vi "Get Rx Label Configuration.vi"(8 "error in":errorcluster, 10 "configuration string":string, 11 "port ref":T1 format="%.0x") -> (0 "error out":errorcluster, 2 "configuration string out":string, 3 "port ref out":T1 format="%.0x")   [LabVIEW 2020, in "Ballard ARINC 429 Hardware Configuration.lvlib"]
uses:
  Ballard ARINC 429 Hardware Configuration.lvlib
  <vilib>/NI VeriStand/Custom Device API/Custom Device Item Ref.ctl
  Constants.vi
  Scripting/Ballard/Ballard ARINC 429 Scripting.lvlib
  <vilib>/NI VeriStand/Custom Device API/Custom Device API.lvlib
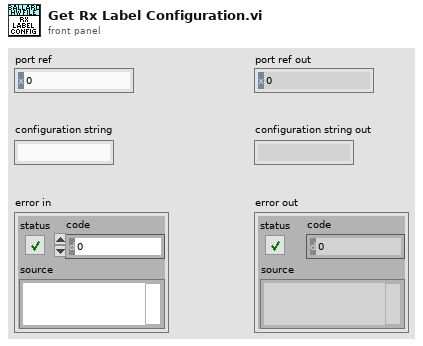
[diagram p1: front panel]
types:
  T1 = typedef "Custom Device API.lvlib/Custom Device Item Ref.ctl" = u64
  T2 = typedef "Label Properties.ctl" = cluster{"label (Dec)":T3, "SDI value":u8, "SDI enabled":bool}
  T3 = typedef "Label.ctl" = u8
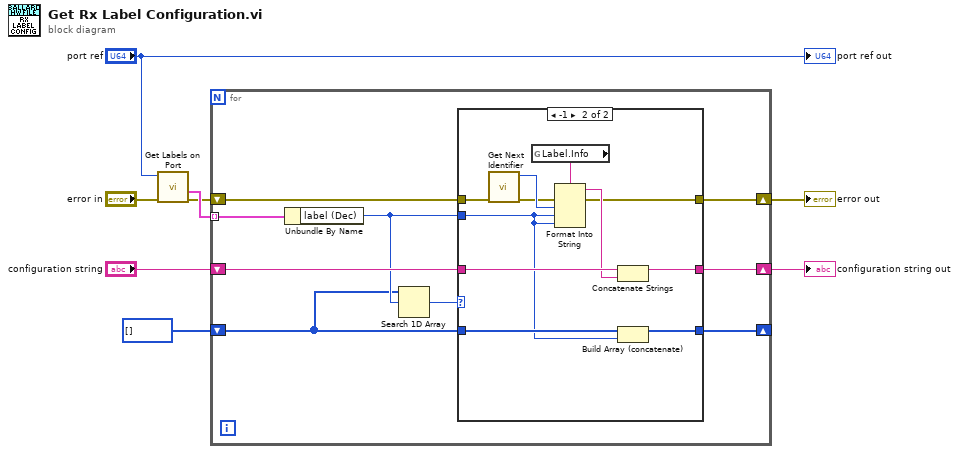
[diagram p0: block diagram]
diagram:
  n1 = call "Get Labels on Port.vi"("error in"="error in", "port in"="port ref") -> ("error out"=w4:errorcluster, "labels properties"=w8:T2[])  [unwired: 6 in, 2 out]
  n2 = for {
    tunnel: w8 -> [w17] mode=indexing
    shift-right: [w16] -> w6
    shift-left: "configuration string" -> [w15]
    shift-right: [w12] -> w3
    shift-left: w4 -> [w9]
    shift-right: [w10] -> _
    shift-left: u8[] [] -> [w11]
    n3 = Unbundle By Name(w17) -> ("label (Dec)"=w14:T3)
    n4 = Search 1D Array(1D array=w11, element=w14) -> (index of element=w13:i32)  [unwired: 1 in]
    n5 = case shown="-1" w13 {
      tunnel: w14 -> [_ w26]
      tunnel: [w20 w30] -> w16
      tunnel: w15 -> [w20 w29]
      tunnel: w9 -> [w19 w24]
      tunnel: [w19 w21] -> w12
      tunnel: w11 -> [w18 w27]
      tunnel: [w18 w25] -> w10
      frame Default {
      }
      frame -1 {
        n6 = call "Get Next Identifier.vi"("error in"=w24) -> ("error out"=w22:errorcluster, "ID"=w23:u32)  [unwired: 9 in]
        n7 = global read "Constants.vi" "Label.Info"() -> (w31:string)
        n8 = Format Into String(format string=w31, error in=w22, w23, w26, w26) -> (resulting string=w28:string, error out=w21:errorcluster)  [unwired: 1 in]
        n9 = Concatenate Strings(w29, w28) -> (w30:string)
        n10 = Build Array (concatenate)(w27, w26) -> (w25:T3[])
      }
    }
  }
  "error out" <- w3
  "configuration string out" <- w6
  "port ref out" <- "port ref"
